vi "Readout Single Channel Cubic Parameters_LV2014.vi"(3 "Data string (without \"Ende\")":string) -> (0 "Channel specific cubic parameters V->T":sgl[][][](array[numeric]) format="%.4e", 1 "Channel specific cubic parameters T->V":sgl[][][](array[numeric]) format="%.4e")   [LabVIEW 2014]
panel:
  # "Fiber"
  # "FBG-Channel"
  # "Parameter"
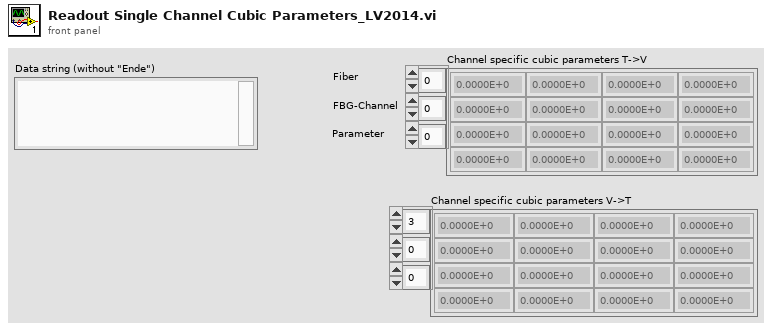
[diagram p1: front panel]
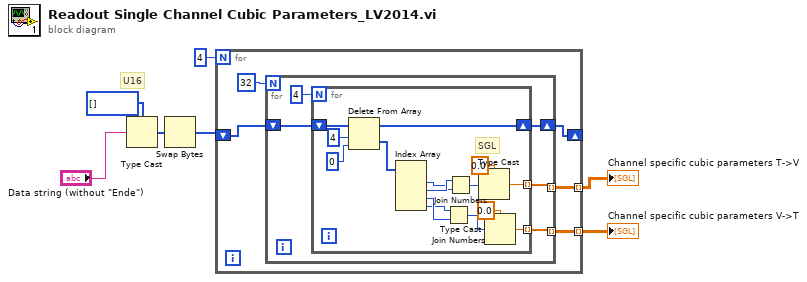
[diagram p0: block diagram]
diagram:
  # "U16"
  n1 = Type Cast(type=u16[] [] ("Angehängtes Array"), x="Data string (without \"Ende\")") -> (*(type *) &x=w4:u16[])
  n2 = Swap Bytes(anything=w4) -> (byte swapped=w2:u16[])
  n3 = for {
    N: 4 -> [_]
    tunnel: [w11] -> w7 mode=indexing
    tunnel: [w10] -> w6 mode=indexing
    shift-right: [w8] -> _
    shift-left: w2 -> [w9]
    n4 = for {
      N: 32 -> [_]
      shift-right: [w16] -> w8
      shift-left: w9 -> [w17]
      tunnel: [w15] -> w10 mode=indexing
      tunnel: [w14] -> w11 mode=indexing
      n5 = for {
        N: 4 -> [_]
        shift-right: [w31] -> w16
        shift-left: w17 -> [w32]
        tunnel: [w23] -> w15 mode=indexing
        tunnel: [w18] -> w14 mode=indexing
        # "SGL"
        n6 = Delete From Array(array=w32, length=4 ("Länge"), index=0 ("Index")) -> (deleted portion=w28:u16[], array with subset deleted=w31:u16[])
        n7 = Index Array(array=w28) -> (element #1=w21:u16, element #2=w22:u16, element #3=w27:u16, element #4=w26:u16)  [unwired: 4 in]
        n8 = Join Numbers(hi=w26, lo=w27) -> ((hi.lo)=w25:u32)
        n9 = Join Numbers(hi=w22, lo=w21) -> ((hi.lo)=w19:u32)
        n10 = Type Cast(type=sgl 0.0, x=w19) -> (*(type *) &x=w18:sgl)
        n11 = Type Cast(type=sgl 0.0, x=w25) -> (*(type *) &x=w23:sgl)
      }
    }
  }
  "Channel specific cubic parameters V->T" <- w6
  "Channel specific cubic parameters T->V" <- w7
